vi "Log.vi"(8 "error in":errorcluster, 10 "Log Entry":T1 {"Time" format="%<%x %.3X>T"}, 11 "Console Logger in":refnum<class "Console Logger.lvclass">) -> (0 "error out":errorcluster, 3 "Console Logger out":refnum<class "Console Logger.lvclass">)   [LabVIEW 2026, in "Console Logger.lvlib" / "Console Logger.lvclass"]
doc: "Log the provided entry."
uses:
  Console Logger.lvclass
  Type Definitions/Log Entry--cluster.ctl
  Console Logger.lvclass/Console Logger.ctl
  <vilib>/Wiresmith Technology/G CLI/CLI Class/CLI.lvclass
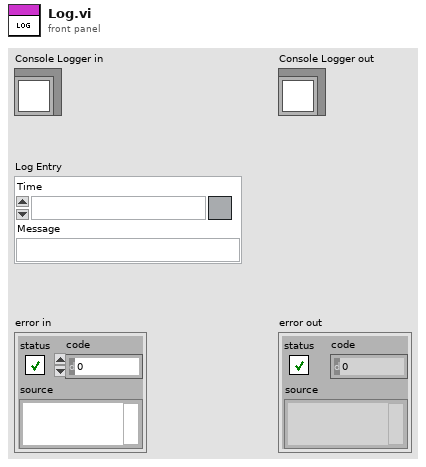
[diagram p1: front panel]
types:
  T1 = typedef "Log Entry--cluster.ctl" = cluster{"Time":timestamp, "Message":string}
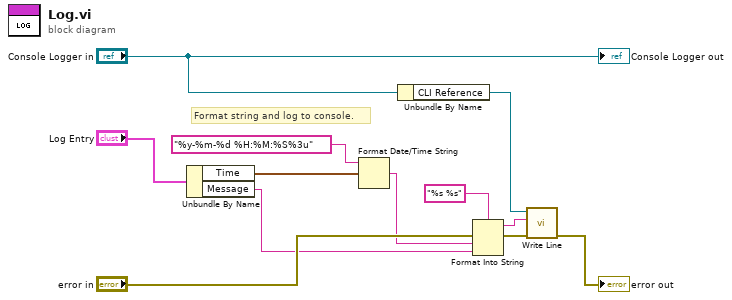
[diagram p0: block diagram]
diagram:
  # "Format string and log to console."
  n1 = Unbundle By Name("Log Entry") -> ("Time"=w8:timestamp, "Message"=w4:string)
  n2 = Format Date/Time String(time format string (%c)="%y-%m-%d %H:%M:%S%3u", seconds (now)=w8) -> (date/time string=w5:string)  [unwired: 1 in]
  n3 = Unbundle By Name("Console Logger in") -> ("CLI Reference"=w2:refnum<class "CLI.lvclass">)
  n4 = Format Into String(format string="%s %s", error in="error in", w5, w4) -> (resulting string=w1:string, error out=w11:errorcluster)  [unwired: 1 in]
  n5 = call <vilib>:"Write Line.vi"("error in (no error)"=w11, "Text to Write"=w1, "CLI in"=w2) -> ("error out"=→"error out":errorcluster)  [unwired: 7 in, 1 out]
  "Console Logger out" <- "Console Logger in"
